vi "Launch UI.vi"(8 "error in (no error)":errorcluster, 11 "Controller In":refnum<class "Controller.lvclass">) -> (0 "error out":errorcluster, 3 "Controller Out":refnum<class "Controller.lvclass">)   [LabVIEW 2026, in "Controller Actor.lvlib" / "Controller.lvclass"]
uses:
  Controller.lvclass
  User Interface/UI.lvclass
  Controller.lvclass/Controller.ctl
  <vilib>/ActorFramework/Actor/Actor.lvclass
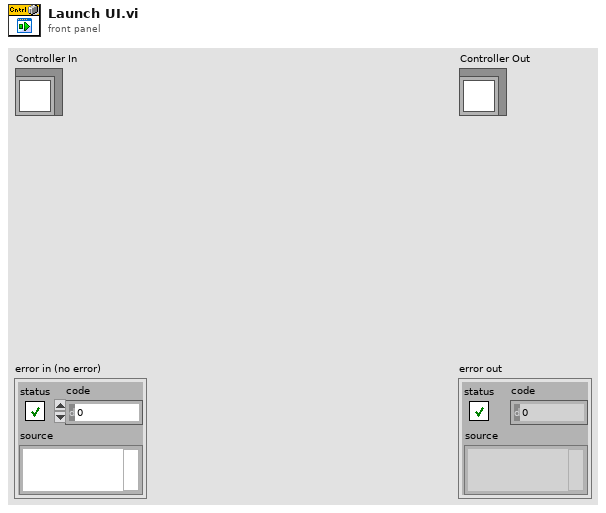
[diagram p1: front panel]
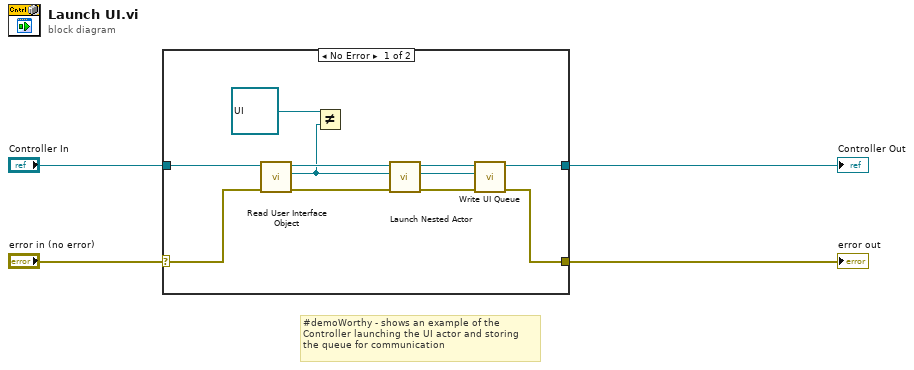
[diagram p0: block diagram]
diagram:
  # "#demoWorthy - shows an example of the \nController launching the UI actor and storing\nthe queue for communication"
  n1 = case shown="No Error" "error in (no error)" {
    selector: "error in (no error)" -> [w13 w17]
    tunnel: [w12 w17] -> w3
    tunnel: [w15 w16] -> w1
    tunnel: "Controller In" -> [w14 w16]
    frame No Error {
      n2 = call "Read User Interface Object.vi"("error in (no error)"=w13, "UI Controller in"=w14) -> ("error out"=w9:errorcluster, "UI.lvclass"=w6:refnum<class "UI.lvclass">, "UI Controller out"=w7:refnum<class "Controller.lvclass">)  [unwired: 7 in]
      n3 = Not Equal?(x=refnum<class "UI.lvclass"> refnum ("Generic UI Actor.lvlib:UI.lvclass"), y=w6) -> ()  [unwired: 1 out]
      n4 = call <vilib>:"Launch Nested Actor.vi"("error in (no error)"=w9, "Nested Actor"=w6, "Caller Actor in"=w7) -> ("error out"=w10:errorcluster, "Nested Actor's Enqueuer"=w11:refnum<class "Message Enqueuer.lvclass">, "Caller Actor out"=w8:refnum<class "Controller.lvclass">)  [unwired: 6 in]
      n5 = call "Write UI Queue.vi"("error in (no error)"=w10, "UI Queue"=w11, "UI Controller in"=w8) -> ("error out"=w12:errorcluster, "UI Controller out"=w15:refnum<class "Controller.lvclass">)  [unwired: 7 in]
    }
    frame Error {
    }
  }
  "error out" <- w3
  "Controller Out" <- w1
